vi "Native_AddForShiftRegister.vi"() -> ()   [LabVIEW 2024]
panel:
  out "error out":errorcluster caption="错误输出"
  out "right_id":u32
  in  "right_id type":u32
  in  "y":u32
  in  "for_id":u32
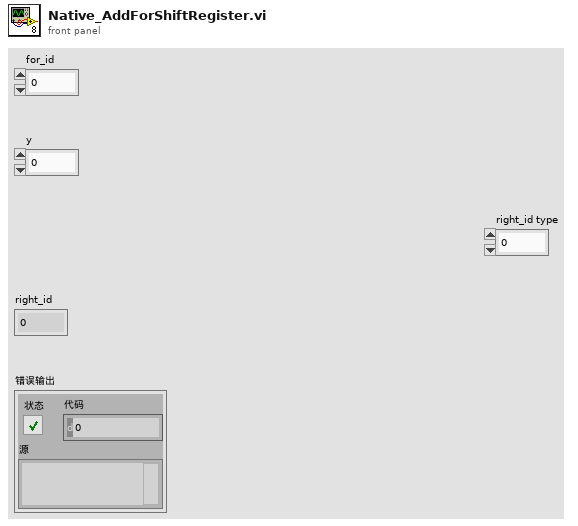
[diagram p1: front panel]
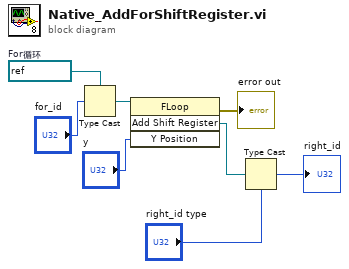
[diagram p0: block diagram]
diagram:
  w7 = refnum<vi> refnum  # For循环
  n1 = Type Cast ("强制类型转换")(type=w7, x="for_id") -> (*(type *) &x=w6:refnum<vi>)
  n2 = invoke class="FLoop" method="Add Shift Register"(reference=w6, "Y Position"="y") -> (error out=→"error out":errorcluster, "Add Shift Register"=w4:refnum<vi>)  [unwired: 2 in, 2 out]
  n3 = Type Cast ("强制类型转换")(type="right_id type", x=w4) -> (*(type *) &x=→"right_id":u32)
